vi "prepareCheckbox.vi"(8 "error in":errorcluster, 9 "current default name":string, 10 "make default Refnum":refnum<vi>, 11 "Current default string ref":refnum<vi>) -> (0 "error out":errorcluster)   [LabVIEW 2023]
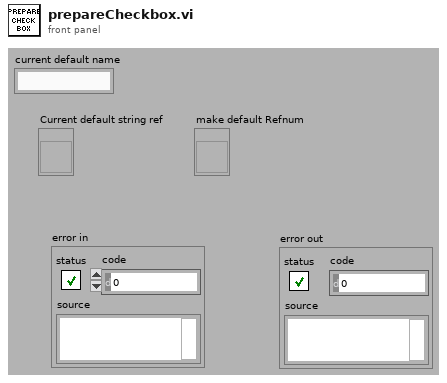
[diagram p1: front panel]
types:
  T1 = enum8{"Enabled", "Disabled", "Disabled and Grayed Out"}
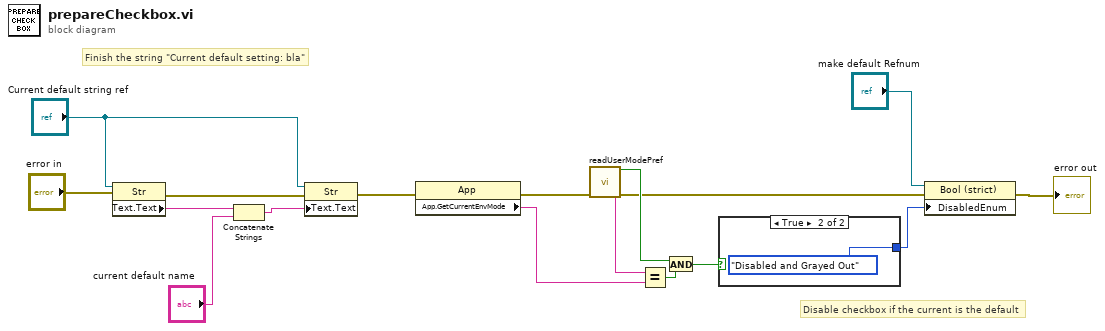
[diagram p0: block diagram]
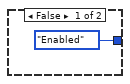
[diagram p2: hidden frame]
diagram:
  # "Finish the string \"Current default setting: bla\""
  # "Disable checkbox if the current is the default"
  n1 = property on="Property Node" class="Str"(reference="Current default string ref", error in="error in") -> (error out=w11:errorcluster, "Text.Text"=w14:string)  [unwired: 1 out]
  n2 = Concatenate Strings(w14, "current default name") -> (w15:string)
  n3 = property on="Property Node" class="Str"(reference="Current default string ref", error in=w11, "Text.Text"=w15) -> (error out=w9:errorcluster)  [unwired: 1 out]
  n4 = property class="App"(error in=w9) -> (error out=w2:errorcluster, "App.GetCurrentEnvMode"=w3:string)  [unwired: 1 in, 1 out]
  n5 = call <resource>:"readUserModePref.vi"("error in"=w2) -> ("found?"=w5:bool, "value read"=w4:string, "error out"=w1:errorcluster)  [unwired: 12 in]
  n6 = Equal?(x=w4, y=w3) -> (x = y?=w7:bool)
  n7 = And(x=w5, y=w7) -> (x .and. y?=w6:bool)
  n8 = case shown="True" w6 {
    tunnel: [T1."Enabled" ("Disabled") T1."Disabled and Grayed Out" ("Disabled")] -> w17
    frame False {
    }
    frame True {
    }
  }
  n9 = property on="Property Node" class="Bool (strict)"(reference="make default Refnum", error in=w1, "DisabledEnum"=w17) -> (error out=→"error out":errorcluster)  [unwired: 1 out]
